vi "start TDMS file.vi"(8 "filename ending":string, 9 "filename prefix":string, 11 "base path":path) -> (3 "tdms file out":refnum<k34>)   [LabVIEW 2025]
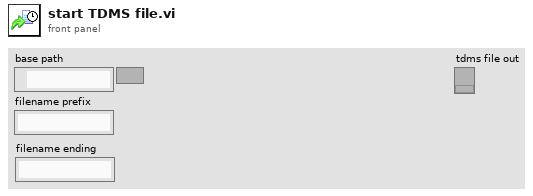
[diagram p1: front panel]
types:
  T1 = enum16{"open", "open or create", "create or replace", "create", "open (read-only)"}
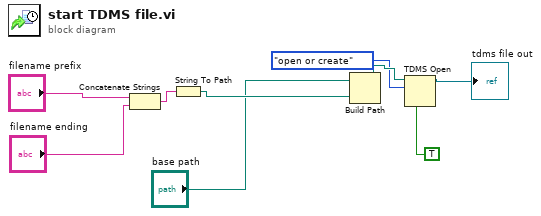
[diagram p0: block diagram]
diagram:
  n1 = Concatenate Strings("filename prefix", "filename ending") -> (w7:string)
  n2 = String To Path(string=w7) -> (path=w8:path)
  n3 = Build Path(base path="base path", name or relative path=w8) -> (appended path=w9:path)
  n4 = TDMS Open(6:TRUE ("disable buffering? (T)"), 10:T1."open or create" ("operation (0:open)"), 11:w9) -> (3:→"tdms file out":refnum<k34>)  [unwired: 4 in, 1 out]
